vi "Omok_Main.vi"() -> ()   [LabVIEW 2026]
doc: "오목 메인 VI (v2). 창 전체가 Picture 하나: 설정 화면(모드/선공/난이도/규칙/게임 시작) -> 게임 화면.\nUI 이벤트 루프(마우스) -> 게임 큐 -> 게임 루프(Context Shift Register, Game_Click/Hover/AI_Move, UI_Render) -> AI 큐 -> AI 작업 루프 -> 게임 큐. 사람 vs AI / 2인 플레이."
panel:
  out "Board":picture
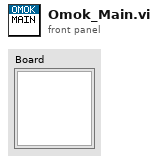
[diagram p1: front panel]
types:
  T1 = cluster{"Screen":enum16{"Settings", "Game"}, "Settings":i32[], "Board":cluster{"Grid":enum8{"Empty", "Black", "White"}[][], "Move History":cluster{"Row":i32, "Col":i32, "Stone":enum8{"Empty", "Black", "White"}}[], "Last Move":cluster{"Row":i32, "Col":i32, "Stone":enum8{"Empty", "Black", "White"}}}, "Status":enum16{"Idle", "Player Turn", "AI Thinking", "Game Over"}, "Game ID":u32, "Player Stone":enum8{"Empty", "Black", "White"}, "Hover":cluster{"Row":i32, "Col":i32, "Stone":enum8{"Empty", "Black", "White"}}, "Hover Button":i32, "Win Line":cluster{"Row":i32, "Col":i32, "Stone":enum8{"Empty", "Black", "White"}}[], "Score 1":i32, "Score 2":i32, "Draws":i32, "Status Text":string, "Status Color":u32}
  T2 = cluster{"Msg":enum16{"Redraw", "Click", "Hover", "AI Move Ready", "Exit"}, "Move":cluster{"Row":i32, "Col":i32, "Stone":enum8{"Empty", "Black", "White"}}, "Game ID":u32, "Point":cluster{"X":i32, "Y":i32}}
  T3 = enum16{"Redraw", "Click", "Hover", "AI Move Ready", "Exit"}
  T4 = cluster{"Grid":enum8{"Empty", "Black", "White"}[][], "AI Stone":enum8{"Empty", "Black", "White"}, "Difficulty":enum8{"Easy", "Normal", "Hard", "Master"}, "Renju":bool, "Game ID":u32, "Stop":bool}
  T5 = cluster{"Left":i32, "Top":i32, "Right":i32, "Bottom":i32}
  T6 = cluster{"Row":i32, "Col":i32, "Stone":enum8{"Empty", "Black", "White"}}
  T7 = cluster{"Grid":enum8{"Empty", "Black", "White"}[][], "Move History":cluster{"Row":i32, "Col":i32, "Stone":enum8{"Empty", "Black", "White"}}[], "Last Move":cluster{"Row":i32, "Col":i32, "Stone":enum8{"Empty", "Black", "White"}}}
  T8 = typedef "LVMouseTypeDef.ctl" = cluster{"Mouse Position":cluster{"X":i32, "Y":i32}, "Mouse Modifiers":cluster{"Button Down":bool, "Shift Mod":bool, "Menu Mod":bool, "Option Mod":bool}}
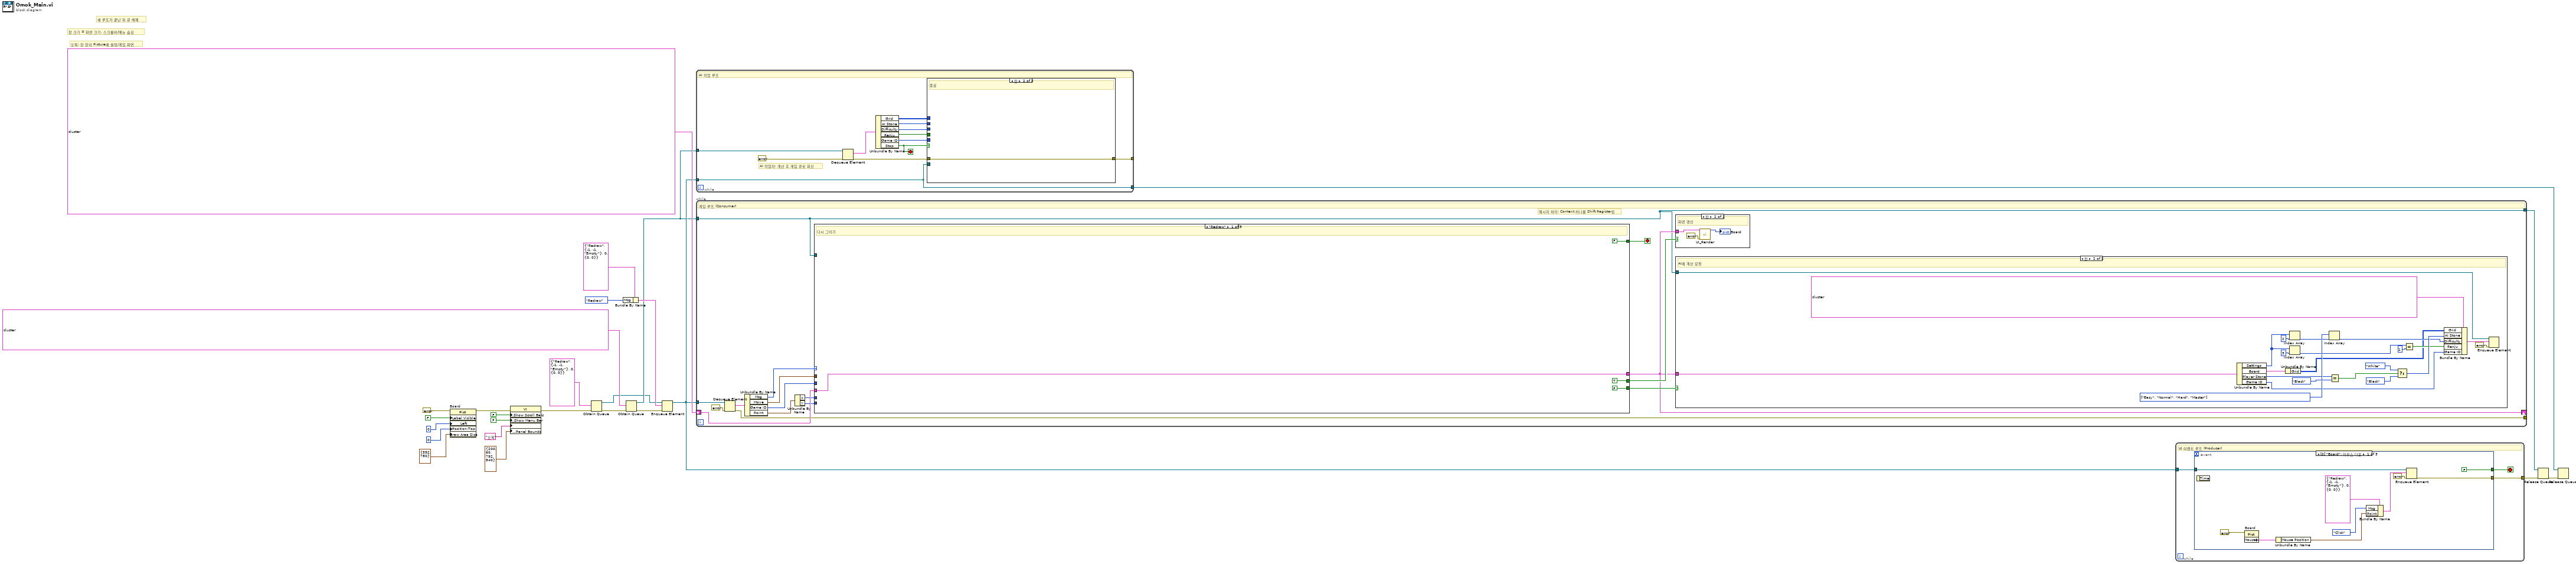
[diagram p0: block diagram]
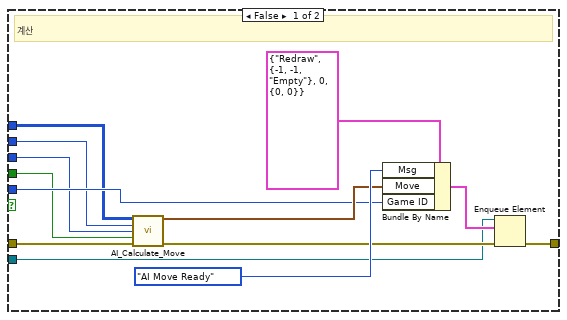
[diagram p2: hidden frame]
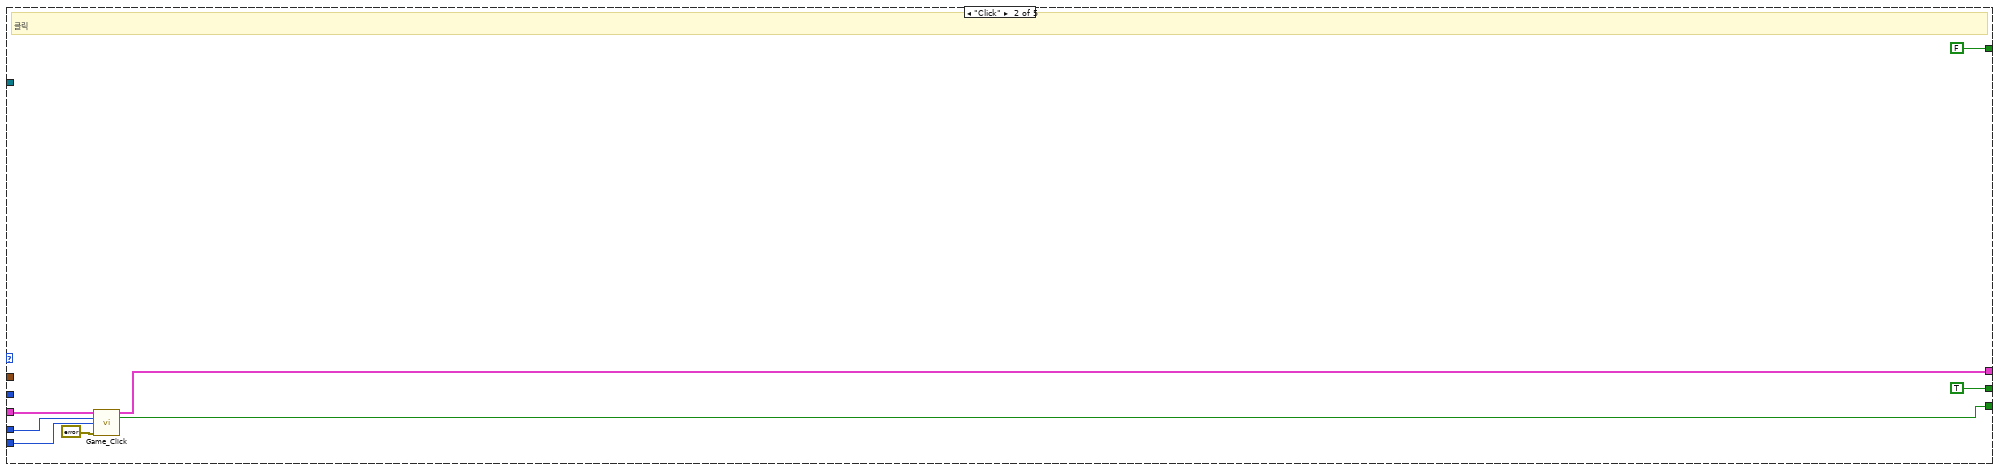
[diagram p5: hidden frame]
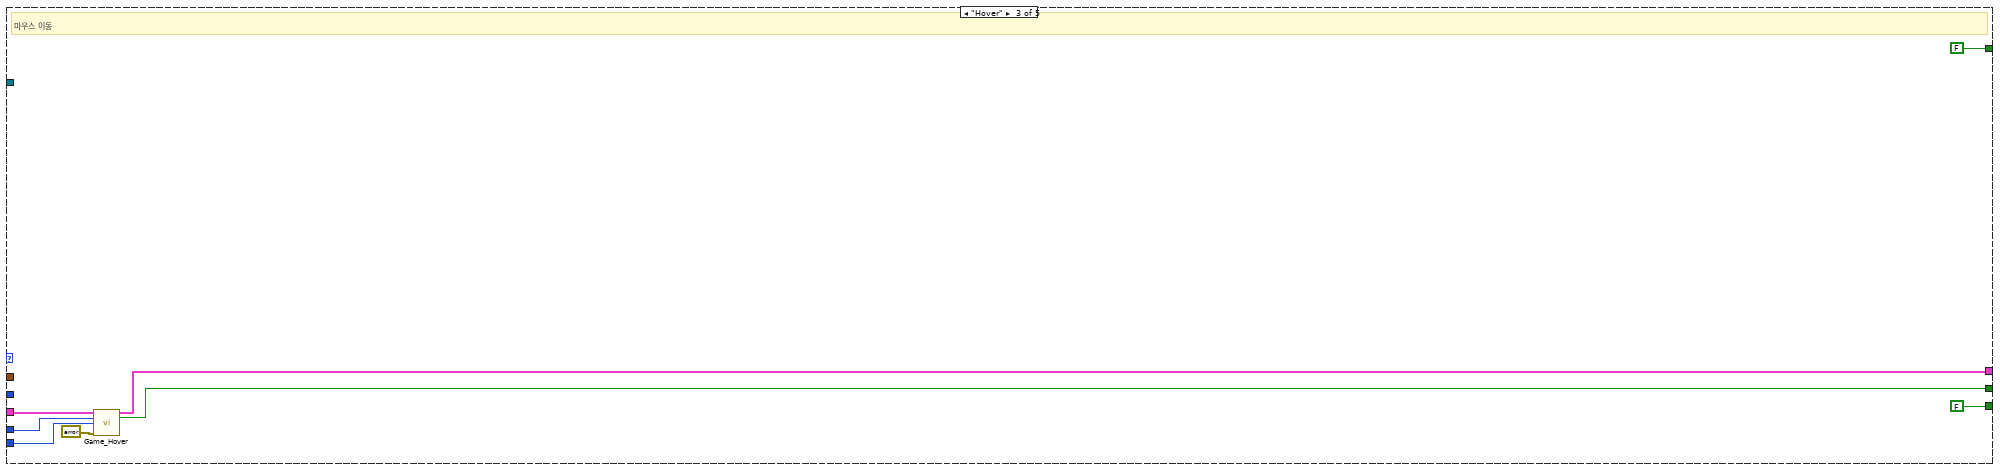
[diagram p6: hidden frame]
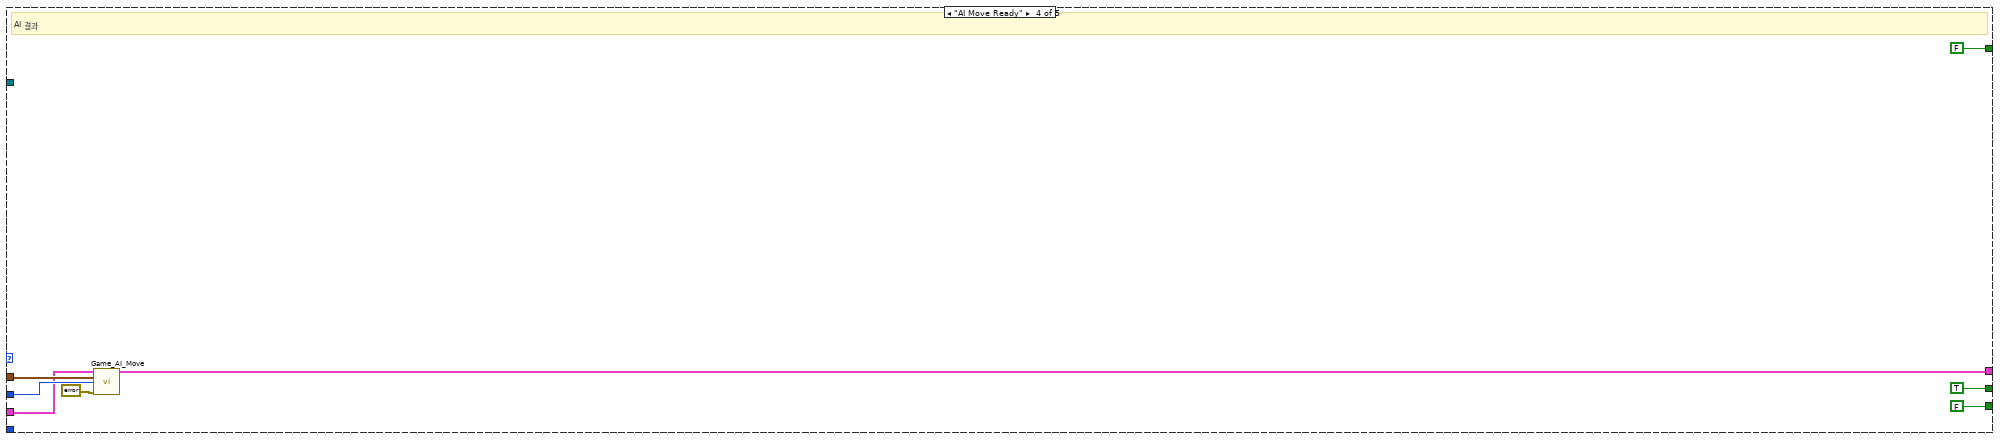
[diagram p7: hidden frame]
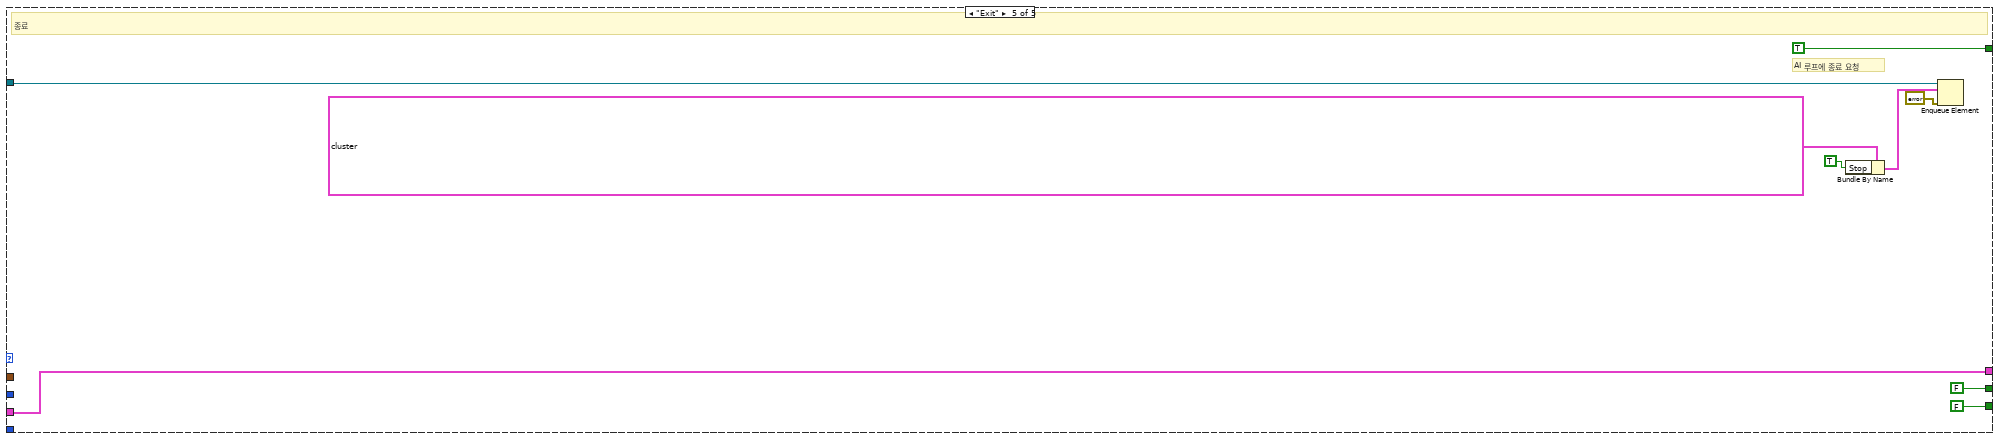
[diagram p8: hidden frame]
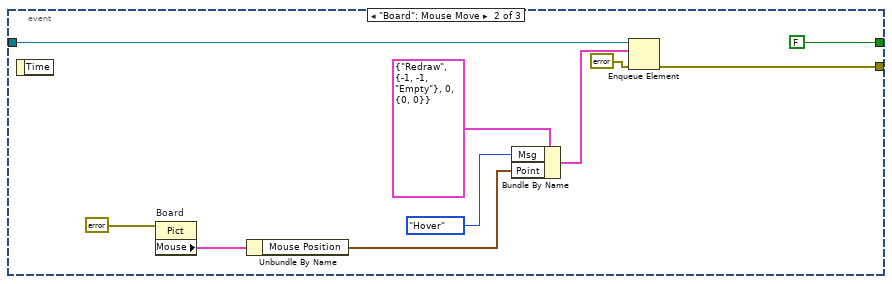
[diagram p9: hidden frame]
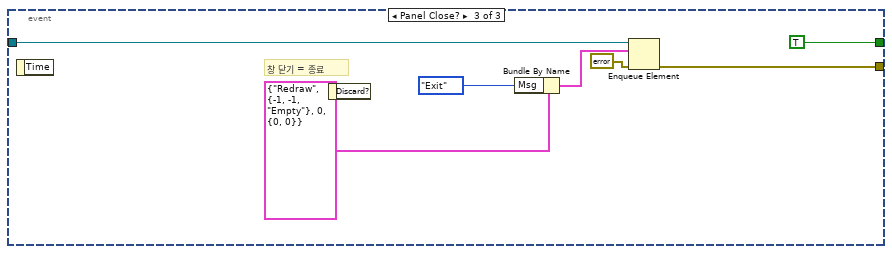
[diagram p10: hidden frame]
diagram:
  # "세 루프가 끝난 뒤 큐 해제"
  # "창 크기 = 화면 크기, 스크롤바/메뉴 숨김"
  # "오목: 한 장의 Picture에 설정/게임 화면"
  n1 = property on="Board" class="Pict"(error in=errorcluster {"status"=FALSE, "code"=0, "source"=""}, "Label.Visible"=FALSE, "Left"=0, "Position:Top"=0, "Draw Area Size"=cluster{"Width":i32, "Height":i32} {"Width"=592, "Height"=780}) -> (error out=w6:errorcluster)  [unwired: 1 in, 1 out]
  n2 = property class="VI"(error in=w6, "Front Panel Window:Show Scroll Bars"=FALSE, "Front Panel Window:Show Menu Bar"=FALSE, "Front Panel Window:Title"="오목", "Front Panel Window:Panel Bounds"=T5 {"Left"=200, "Top"=60, "Right"=792, "Bottom"=840}) -> (error out=w11:errorcluster)  [unwired: 1 in, 1 out]
  n3 = Obtain Queue(element data type=T2 {"Msg"=enum."Redraw", "Move"={"Row"=-1, "Col"=-1, "Stone"=enum."Empty"}, "Game ID"=0, "Point"={"X"=0, "Y"=0}}, error in (no error)=w11) -> (queue out=w13:refnum<queue>, error out=w14:errorcluster)  [unwired: 3 in, 1 out]
  n4 = Bundle By Name(cluster=T2 {"Msg"=enum."Redraw", "Move"={"Row"=-1, "Col"=-1, "Stone"=enum."Empty"}, "Game ID"=0, "Point"={"X"=0, "Y"=0}}, "Msg"=T3."Redraw") -> (w20:T2)
  n5 = Obtain Queue(element data type=T4 {"Grid"=array15x15[225 elements], "AI Stone"=enum."White", "Difficulty"=enum."Normal", "Renju"=TRUE, "Game ID"=0, "Stop"=FALSE}, error in (no error)=w14) -> (queue out=w16:refnum<queue>, error out=w17:errorcluster)  [unwired: 3 in, 1 out]
  n6 = Enqueue Element(queue=w13, element=w20, error in (no error)=w17) -> (queue out=w21:refnum<queue>)  [unwired: 1 in, 2 out]
  n7 = while {
    tunnel: w16 -> [w27]
    tunnel: w21 -> [w28]
    tunnel: [w28] -> w25
    tunnel: [w38] -> _
    stop <- w37 stop-if-true
    # "AI 작업자: 계산 후 게임 큐로 회신"
    # "AI 작업 루프"
    n8 = Dequeue Element(queue=w27, error in (no error)=errorcluster {"status"=FALSE, "code"=0, "source"=""}) -> (element=w30:T4, error out=w31:errorcluster)  [unwired: 1 in, 2 out]
    n9 = Unbundle By Name(w30) -> ("Grid"=w32:enum8{"Empty", "Black", "White"}[][], "AI Stone"=w33:enum8{"Empty", "Black", "White"}, "Difficulty"=w34:enum8{"Easy", "Normal", "Hard", "Master"}, "Renju"=w35:bool, "Game ID"=w36:u32, "Stop"=w37:bool)
    n10 = case shown="참" w37 {
      tunnel: w28 -> [w44 _]
      tunnel: w31 -> [w45 w52]
      tunnel: w32 -> [w39 _]
      tunnel: w33 -> [w40 _]
      tunnel: w34 -> [w41 _]
      tunnel: w35 -> [w42 _]
      tunnel: w36 -> [w43 _]
      tunnel: [w51 w52] -> w38
      frame False {
        # "계산"
        n11 = call "AI_Calculate_Move.vi"("Grid"=w39, "AI Stone"=w40, "Difficulty"=w41, "Renju"=w42, "error in"=w45) -> ("Move"=w46:T6, "error out"=w47:errorcluster)  [unwired: 7 in, 2 out]
        n12 = Bundle By Name(cluster=T2 {"Msg"=enum."Redraw", "Move"={"Row"=-1, "Col"=-1, "Stone"=enum."Empty"}, "Game ID"=0, "Point"={"X"=0, "Y"=0}}, "Msg"=T3."AI Move Ready", "Move"=w46, "Game ID"=w43) -> (w50:T2)
        n13 = Enqueue Element(queue=w44, element=w50, error in (no error)=w47) -> (error out=w51:errorcluster)  [unwired: 1 in, 2 out]
      }
      frame True {
        # "종료"
      }
    }
  }
  n14 = while {
    shift-right: [w65] -> _
    shift-left: T1 {"Screen"=enum."Settings", "Settings"=[0, 0, 1, 1], "Board"={"Grid"=array15x15[225 elements], "Move History"=[], "Last Move"={"Row"=-1, "Col"=-1, "Stone"=enum."Empty"}}, "Status"=enum."Idle", "Game ID"=0, "Player Stone"=enum."Black", "Hover"={"Row"=-1, "Col"=-1, "Stone"=enum."Empty"}, "Hover Button"=-1, "Win Line"=[], "Score 1"=0, "Score 2"=0, "Draws"=0, "Status Text"="", "Status Color"=0} -> [w64]
    tunnel: w16 -> [w54]
    tunnel: w21 -> [w53]
    tunnel: [w54] -> w24
    tunnel: [w57] -> _
    stop <- w68 stop-if-true
    # "메시지 처리: Context 하나를 Shift Register로"
    # "게임 루프 (Consumer)"
    n15 = Dequeue Element(queue=w53, error in (no error)=errorcluster {"status"=FALSE, "code"=0, "source"=""}) -> (element=w56:T2, error out=w57:errorcluster)  [unwired: 1 in, 2 out]
    n16 = Unbundle By Name(w56) -> ("Msg"=w58:T3, "Move"=w59:T6, "Game ID"=w60:u32, "Point"=w61:cluster{"X":i32, "Y":i32})
    n17 = Unbundle By Name(w61) -> ("X"=w62:i32, "Y"=w63:i32)
    n18 = case shown="\"Redraw\"" w58 {
      tunnel: [FALSE w104 FALSE FALSE FALSE] -> w66
      tunnel: [TRUE TRUE w112 TRUE FALSE] -> w67
      tunnel: [FALSE FALSE FALSE FALSE TRUE] -> w68
      tunnel: w64 -> [w95 w99 w107 w115 w123]
      tunnel: [w95 w103 w111 w119 w123] -> w65
      tunnel: w54 -> [_ _ _ _ w124]
      tunnel: w59 -> [_ _ _ w116 _]
      tunnel: w60 -> [_ _ _ w117 _]
      tunnel: w62 -> [_ w100 w108 _ _]
      tunnel: w63 -> [_ w101 w109 _ _]
      frame "Redraw" {
        # "다시 그리기"
      }
      frame "Click" {
        # "클릭"
        n19 = call "Game_Click.vi"("Context"=w99, "X"=w100, "Y"=w101, "error in"=errorcluster {"status"=FALSE, "code"=0, "source"=""}) -> ("Context out"=w103:T1, "Need AI"=w104:bool)  [unwired: 9 in, 1 out]
      }
      frame "Hover" {
        # "마우스 이동"
        n20 = call "Game_Hover.vi"("Context"=w107, "X"=w108, "Y"=w109, "error in"=errorcluster {"status"=FALSE, "code"=0, "source"=""}) -> ("Context out"=w111:T1, "Changed"=w112:bool)  [unwired: 9 in, 1 out]
      }
      frame "AI Move Ready" {
        # "AI 결과"
        n21 = call "Game_AI_Move.vi"("Context"=w115, "Move"=w116, "Game ID"=w117, "error in"=errorcluster {"status"=FALSE, "code"=0, "source"=""}) -> ("Context out"=w119:T1)  [unwired: 10 in, 1 out]
      }
      frame "Exit" {
        # "AI 루프에 종료 요청"
        # "종료"
        n22 = Bundle By Name(cluster=T4 {"Grid"=array15x15[225 elements], "AI Stone"=enum."White", "Difficulty"=enum."Normal", "Renju"=TRUE, "Game ID"=0, "Stop"=FALSE}, "Stop"=TRUE) -> (w127:T4)
        n23 = Enqueue Element(queue=w124, element=w127, error in (no error)=errorcluster {"status"=FALSE, "code"=0, "source"=""}) -> ()  [unwired: 1 in, 3 out]
      }
    }
    n24 = case shown="참" w67 {
      tunnel: w65 -> [_ w69]
      frame False {
        # "변화 없음"
      }
      frame True {
        # "화면 갱신"
        n25 = call "UI_Render.vi"("Context"=w69, "error in"=errorcluster {"status"=FALSE, "code"=0, "source"=""}) -> ("Picture"=→"Board":picture)  [unwired: 12 in, 1 out]
      }
    }
    n26 = case shown="참" w66 {
      tunnel: w65 -> [_ w72]
      tunnel: w54 -> [_ w73]
      frame False {
      }
      frame True {
        w79 = enum8{"Easy", "Normal", "Hard", "Master"}[] [enum."Easy", enum."Normal", enum."Hard", enum."Master"] items=["Easy", "Normal", "Hard", "Master"] ("Difficulties")
        # "AI에 계산 요청"
        n27 = Unbundle By Name(w72) -> ("Settings"=w74:i32[], "Board"=w75:T7, "Player Stone"=w76:enum8{"Empty", "Black", "White"}, "Game ID"=w77:u32)
        n28 = Unbundle By Name(w75) -> ("Grid"=w78:enum8{"Empty", "Black", "White"}[][])
        n29 = Index Array(array=w74, index=2) -> (element=w81:i32)
        n30 = Index Array(array=w74, index=3) -> (element=w84:i32)
        n31 = Index Array(array=w79, index=w81) -> (element=w82:enum8{"Easy", "Normal", "Hard", "Master"})
        n32 = Equal?(x=w76, y=enum8{"Empty", "Black", "White"}."Black") -> (x = y?=w88:bool)
        n33 = Select(t=enum8{"Empty", "Black", "White"}."White", s=w88, f=enum8{"Empty", "Black", "White"}."Black") -> (s? t:f=w91:enum8{"Empty", "Black", "White"})
        n34 = Equal?(x=w84, y=1) -> (x = y?=w86:bool)
        n35 = Bundle By Name(cluster=T4 {"Grid"=array15x15[225 elements], "AI Stone"=enum."White", "Difficulty"=enum."Normal", "Renju"=TRUE, "Game ID"=0, "Stop"=FALSE}, "Grid"=w78, "AI Stone"=w91, "Difficulty"=w82, "Renju"=w86, "Game ID"=w77) -> (w93:T4)
        n36 = Enqueue Element(queue=w73, element=w93, error in (no error)=errorcluster {"status"=FALSE, "code"=0, "source"=""}) -> ()  [unwired: 1 in, 3 out]
      }
    }
  }
  n37 = while {
    tunnel: w21 -> [w132]
    tunnel: [w134] -> w22
    stop <- w133 stop-if-true
    # "UI 이벤트 루프 (Producer)"
    n38 = event shown="[0] \"Board\": 마우스 다운" {
      selector: _ -> [_ _ _]
      dyn-events: _ -> [_ _ _]
      timeout: _ -> [_ _ _]
      tunnel: [FALSE FALSE TRUE] -> w133
      tunnel: w132 -> [w135 w145 w155]
      tunnel: [w143 w153 w160] -> w134
      event "Board": Mouse Down {
        n39 = event-data() -> ()  [unwired: 1 in, 1 out]
        n40 = property on="Board" class="Pict"(error in=errorcluster {"status"=FALSE, "code"=0, "source"=""}) -> ("Mouse"=w137:T8)  [unwired: 1 in, 2 out]
        n41 = Unbundle By Name(w137) -> ("Mouse Position"=w138:cluster{"X":i32, "Y":i32})
        n42 = Bundle By Name(cluster=T2 {"Msg"=enum."Redraw", "Move"={"Row"=-1, "Col"=-1, "Stone"=enum."Empty"}, "Game ID"=0, "Point"={"X"=0, "Y"=0}}, "Msg"=T3."Click", "Point"=w138) -> (w141:T2)
        n43 = Enqueue Element(queue=w135, element=w141, error in (no error)=errorcluster {"status"=FALSE, "code"=0, "source"=""}) -> (error out=w143:errorcluster)  [unwired: 1 in, 2 out]
      }
      event "Board": Mouse Move {
        n44 = event-data() -> ()  [unwired: 1 in, 1 out]
        n45 = property on="Board" class="Pict"(error in=errorcluster {"status"=FALSE, "code"=0, "source"=""}) -> ("Mouse"=w147:T8)  [unwired: 1 in, 2 out]
        n46 = Unbundle By Name(w147) -> ("Mouse Position"=w148:cluster{"X":i32, "Y":i32})
        n47 = Bundle By Name(cluster=T2 {"Msg"=enum."Redraw", "Move"={"Row"=-1, "Col"=-1, "Stone"=enum."Empty"}, "Game ID"=0, "Point"={"X"=0, "Y"=0}}, "Msg"=T3."Hover", "Point"=w148) -> (w151:T2)
        n48 = Enqueue Element(queue=w145, element=w151, error in (no error)=errorcluster {"status"=FALSE, "code"=0, "source"=""}) -> (error out=w153:errorcluster)  [unwired: 1 in, 2 out]
      }
      event Panel Close? {
        # "창 닫기 = 종료"
        n49 = event-data() -> ()  [unwired: 1 in, 1 out]
        n50 = event-data() -> ()  [unwired: 2 in, 1 out]
        n51 = Bundle By Name(cluster=T2 {"Msg"=enum."Redraw", "Move"={"Row"=-1, "Col"=-1, "Stone"=enum."Empty"}, "Game ID"=0, "Point"={"X"=0, "Y"=0}}, "Msg"=T3."Exit") -> (w158:T2)
        n52 = Enqueue Element(queue=w155, element=w158, error in (no error)=errorcluster {"status"=FALSE, "code"=0, "source"=""}) -> (error out=w160:errorcluster)  [unwired: 1 in, 2 out]
      }
    }
  }
  n53 = Release Queue(queue=w24, error in (no error)=w22) -> (error out=w26:errorcluster)  [unwired: 1 in, 2 out]
  n54 = Release Queue(queue=w25, error in (no error)=w26) -> ()  [unwired: 1 in, 3 out]
